vi "Variant_AppendElementToCluster.vi"(7 "Path":string, 9 "Element name":string, 10 "Element":variant, 11 "Data in":variant) -> (3 "Data out":variant)   [LabVIEW 2013, in "OpenVariant.lvlib"]
uses:
  OpenVariant.lvlib
  TypeDescriptor/TypeDescriptor_GetName.vi
  TypeDescriptor/TypeDescriptor_GetPString.vi
  TypeDescriptor/TypeDescriptor_SetName.vi
  <vilib>/Utility/GetType.llb/TD_Create Cluster.vi
  TypeDescriptor/VariantToDescriptorElements.vi
  Conversions/OpenConvert.lvlib
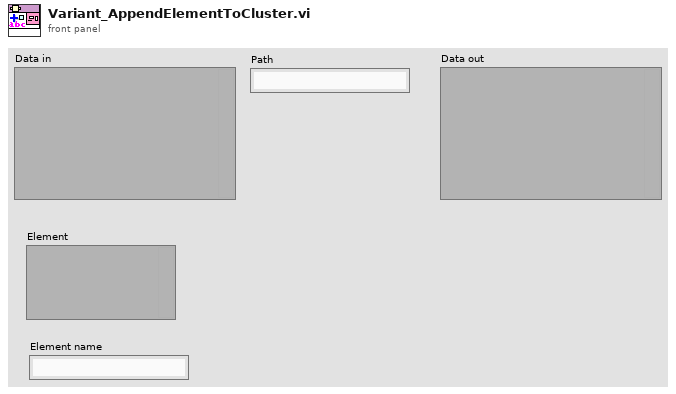
[diagram p1: front panel]
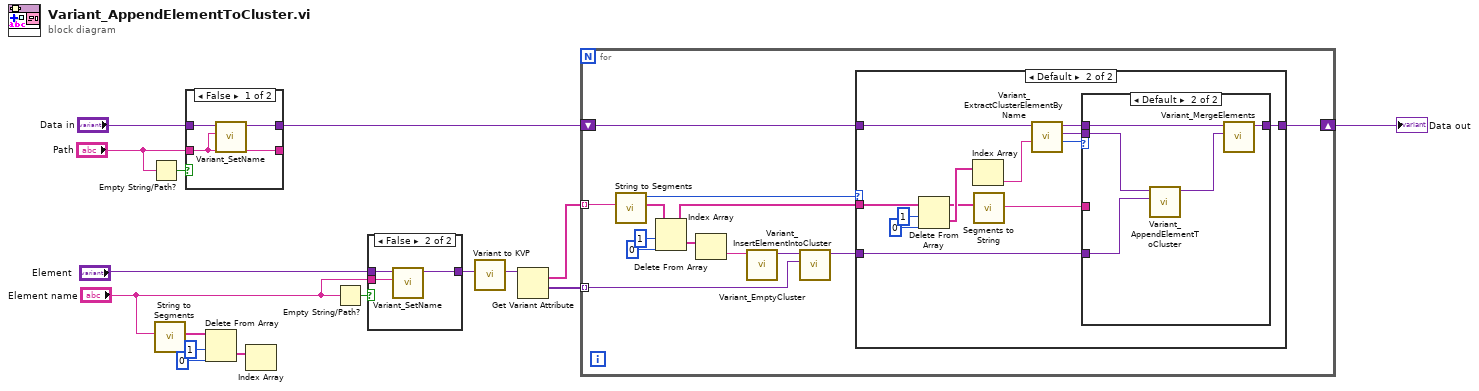
[diagram p0: block diagram]
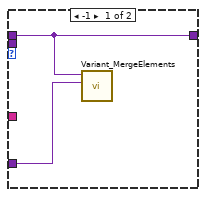
[diagram p3: hidden frame]
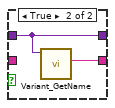
[diagram p5: hidden frame]
diagram:
  n1 = Empty String/Path?(string/path="Path") -> (empty?=w14:bool)
  n2 = call "String to Segments.vi"("String"="Element name") -> ("Segments"=w1:string[])  [unwired: 9 in, 1 out]
  n3 = case shown="False" w14 {
    tunnel: "Path" -> [w17 _]
    tunnel: "Data in" -> [w19 w21]
    tunnel: [w18 w21] -> w8
    tunnel: [w17 w20] -> _
    frame False {
      n4 = call "Variant_SetName.vi"("Name"=w17, "Variant"=w19) -> ("Named Variant"=w18:variant)  [unwired: 9 in]
    }
    frame True {
      n5 = call "Variant_GetName.vi"("Variant"=w21) -> ("Name"=w20:string)  [unwired: 8 in, 2 out]
    }
  }
  n6 = Delete From Array(array=w1, length=1, index=0) -> (deleted portion=w4:string[])  [unwired: 1 out]
  n7 = Index Array(array=w4) -> ()  [unwired: 1 in, 1 out]
  n8 = Empty String/Path?(string/path="Element name") -> (empty?=w12:bool)
  n9 = case shown="False" w12 {
    tunnel: "Element name" -> [_ w23]
    tunnel: "Element" -> [w22 w25]
    tunnel: [w22 w24] -> w6
    frame True {
    }
    frame False {
      n10 = call "Variant_SetName.vi"("Name"=w23, "Variant"=w25) -> ("Named Variant"=w24:variant)  [unwired: 9 in]
    }
  }
  n11 = call "Variant to KVP.vi"("Variant"=w6) -> ("KVP Dictionary"=w11:variant)  [unwired: 10 in]
  n12 = Get Variant Attribute(Variant=w11) -> (names=w7:string[], values=w10:variant[])  [unwired: 3 in, 2 out]
  n13 = for {
    tunnel: w7 -> [w37] mode=indexing
    tunnel: w10 -> [w27] mode=indexing
    shift-right: [w36] -> w9
    shift-left: w8 -> [w38]
    n14 = call "String to Segments.vi"("String"=w37) -> ("Segments"=w32:string[], "Nb segments"=w35:i32)  [unwired: 9 in]
    n15 = Delete From Array(array=w32, length=1, index=0) -> (deleted portion=w30:string[], array with subset deleted=w31:string[])
    n16 = Index Array(array=w30) -> (element=w28:string)  [unwired: 1 in]
    n17 = call "Variant_EmptyCluster.vi"("Cluster Name"=w28) -> ("Empty Cluster"=w29:variant)  [unwired: 10 in]
    n18 = call "Variant_InsertElementIntoCluster.vi"("Element"=w27, "Cluster in"=w29) -> ("Cluster out"=w26:variant)  [unwired: 9 in]
    n19 = case shown="Default" w35 {
      tunnel: w38 -> [w39 w52]
      tunnel: [w39 w43] -> w36
      tunnel: w31 -> [_ w51]
      tunnel: w26 -> [_ w45]
      frame 0 {
      }
      frame Default {
        n20 = Delete From Array(array=w51, length=1, index=0) -> (deleted portion=w48:string[], array with subset deleted=w47:string[])
        n21 = Index Array(array=w48) -> (element=w42:string)  [unwired: 1 in]
        n22 = call "Segments to String.vi"("Segments"=w47) -> ("String"=w40:string)  [unwired: 10 in]
        n23 = call "Variant_ExtractClusterElementByName.vi"("name"=w42, "Cluster"=w52) -> ("index"=w41:i32, "Element"=w46:variant, "Cluster dup"=w44:variant)  [unwired: 7 in]
        n24 = case shown="Default" w41 {
          tunnel: w46 -> [_ w59]
          tunnel: w45 -> [w54 w58]
          tunnel: w44 -> [w53 w56]
          tunnel: [w53 w55] -> w43
          tunnel: w40 -> [_ _]
          frame -1 {
            n25 = call "Variant_MergeElements.vi"("New Element(s)"=w54, "Original Element(s)"=w53) -> ()  [unwired: 9 in, 1 out]
          }
          frame Default {
            n26 = call "Variant_AppendElementToCluster.vi"("Element"=w58, "Data in"=w59) -> ("Data out"=w57:variant)  [unwired: 9 in]
            n27 = call "Variant_MergeElements.vi"("New Element(s)"=w57, "Original Element(s)"=w56) -> ("Merged Elements"=w55:variant)  [unwired: 9 in]
          }
        }
      }
    }
  }
  "Data out" <- w9
